vi "New LINX-PCA9685 PWM.vi"(8 "error in (no error)":errorcluster, 10 "I2C Slave Address (0x40)":u8=64 format="%.0x", 11 "I2C":refnum<class "LINX I2C.lvclass">) -> (0 "error out":errorcluster, 3 "LINX-PCA9865 PWM out":refnum<class "LINX-PCA9685 PWM.lvclass">)   [LabVIEW 2020, in "LINX-PCA9685 PWM.lvclass"]
doc: "Creates a new instance of the PCA9685 from the configured I2C channel."
uses:
  LINX-PCA9685 PWM.lvclass
  LINX I2C/LINX I2C.lvclass
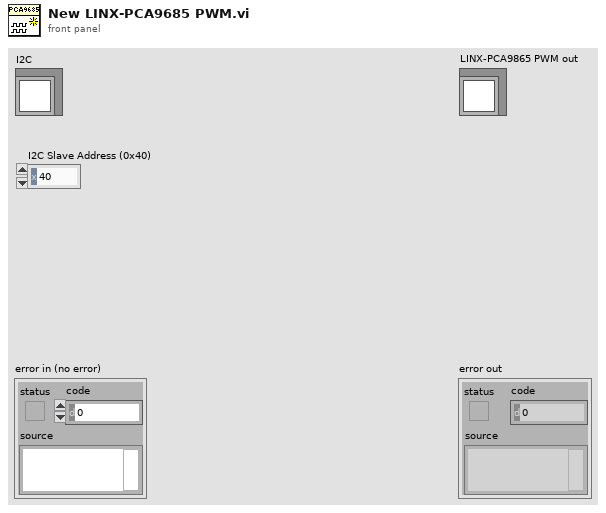
[diagram p1: front panel]
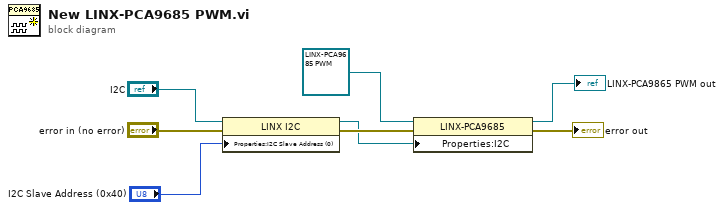
[diagram p0: block diagram]
diagram:
  n1 = property class="LINX I2C"(reference="I2C", error in="error in (no error)", "Properties:I2C Slave Address (0)"="I2C Slave Address (0x40)") -> (reference out=w1:refnum<class "LINX I2C.lvclass">, error out=w4:errorcluster)
  n2 = property class="LINX-PCA9685"(reference=refnum<class "LINX-PCA9685 PWM.lvclass"> refnum ("LINX-PCA9865 PWM in"), error in=w4, "Properties:I2C"=w1) -> (reference out=→"LINX-PCA9865 PWM out":refnum<class "LINX-PCA9685 PWM.lvclass">, error out=→"error out":errorcluster)
